vi "query LTE Uplink Channel Number.vi"(8 "error in (no error)":errorcluster, 9 "UL Channel Arguments":T2, 11 "Anritsu Call Box_Implement in":refnum<class "Anritsu Call Box_Implement.lvclass">) -> (0 "error out":errorcluster, 2 "UL Channel Info":T1, 3 "Anritsu Call Box_Implement out":refnum<class "Anritsu Call Box_Implement.lvclass">)   [LabVIEW 2023, in "ANRITSU Call Box.lvlib" / "Anritsu Call Box_Implement.lvclass"]
uses:
  Anritsu Call Box_Implement.lvclass
  Anritsu Call Box_Implement.lvclass/Anritsu Call Box_Implement.ctl
  LTE/LTE.lvclass
  Type Definition/LTE Uplink Channel Number Target.ctl
  ANRITSU Call Box.lvlib
  Type Definition/LTE Uplink Channel Number Info.ctl
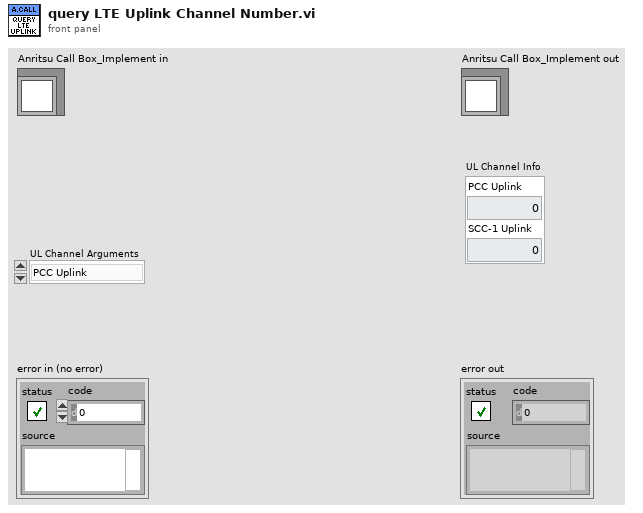
[diagram p1: front panel]
types:
  T1 = typedef "ANRITSU Call Box.lvlib/LTE Uplink Channel Number Info.ctl" = cluster{"PCC Uplink":i32, "SCC-1 Uplink":i32}
  T2 = typedef "ANRITSU Call Box.lvlib/LTE Uplink Channel Number Target.ctl" = enum16{"PCC Uplink", "SCC-1 Uplink", "All"}
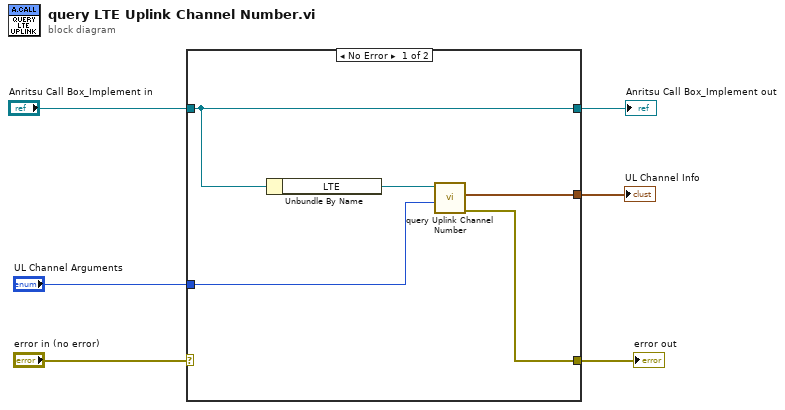
[diagram p0: block diagram]
diagram:
  n1 = case shown="No Error" "error in (no error)" {
    selector: "error in (no error)" -> [_ w12]
    tunnel: "Anritsu Call Box_Implement in" -> [w11 w13]
    tunnel: [w11 w13] -> w5
    tunnel: [w8 w12] -> w3
    tunnel: "UL Channel Arguments" -> [w9 _]
    tunnel: [w7 _] -> w1
    frame No Error {
      n2 = Unbundle By Name(w11) -> ("LTE"=w10:refnum<class "LTE.lvclass">)
      n3 = call "query Uplink Channel Number.vi"("UL Channel Arguments"=w9, "LTE in"=w10) -> ("error out"=w8:errorcluster, "UL Channel Info"=w7:T1)  [unwired: 7 in, 1 out]
    }
    frame Error {
    }
  }
  "error out" <- w3
  "Anritsu Call Box_Implement out" <- w5
  "UL Channel Info" <- w1
